vi "Func Globals xxx.vi"() -> ()   [LabVIEW 2021]
doc: "::: CalcExpress Toolkit :::\nCopyright (c) 2000-2026 Konstantin Shifershteyn. All rights reserved."
panel:
  in  "Gen FuncVI RT errors":bool
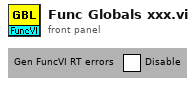
[diagram p1: front panel]
diagram:
